vi "Main.vi"(9 "Test Titel":string, 10 "Cluster 2":T1={"Test Titel"="", "Test Type "="", "Project Number"="NA", "Unit Family"="Package", "Test Procedure #"="", "Data Collection Rate (HZ)"="", "Cluster"={" Pressure /Torque/ LVDT"={"Boolean"=FALSE, "Boolean 2"=FALSE, "Boolean 3"=FALSE, "Boolean 4"=FALSE, "Boolean 5"=FALSE, "Boolean 6"=FALSE, "Boolean 7"=FALSE, "Boolean 8"=FALSE}, "Name of Channel"={"ch1"="", "ch1 2"="", "ch1 3"="", "ch1 4"="", "ch1 5"="", "ch1 6"="", "ch1 7"="", "ch1 8"=""}, "Create New Test"=FALSE, "Name of Channel 2"={"ch1"="", "ch1 2"="", "ch1 3"="", "ch1 4"="", "ch1 5"="", "ch1 6"="", "ch1 7"="", "ch1 8"="", "ch1 9"="", "ch1 10"="", "ch1 11"="", "ch1 12"="", "ch1 13"="", "ch1 14"="", "ch1 15"=""}, "MOD1 ThermoCouple"={"Boolean"=FALSE, "Boolean 2"=FALSE, "Boolean 3"=FALSE, "Boolean 4"=FALSE, "Boolean 5"=FALSE, "Boolean 6"=FALSE, "Boolean 7"=FALSE, "Boolean 8"=FALSE, "Boolean 9"=FALSE, "Boolean 10"=FALSE, "Boolean 11"=FALSE, "Boolean 12"=FALSE, "Boolean 13"=FALSE, "Boolean 14"=FALSE, "Boolean 15"=FALSE, "Boolean 16"=FALSE}, "Internal SFI sensor number"={"ch1"="", "ch1 2"="", "ch1 3"="", "ch1 4"="", "ch1 5"="", "ch1 6"="", "ch1 7"="", "ch1 8"=""}, "Internal SFI sensor number"={"ch1"="", "ch1 2"="", "ch1 3"="", "ch1 4"="", "ch1 5"="", "ch1 6"="", "ch1 7"="", "ch1 8"="", "ch1 9"="", "ch1 10"="", "ch1 11"="", "ch1 12"="", "ch1 13"="", "ch1 14"="", "ch1 15"=""}}, "Sensor Serial Num"="", "Calibration Due"=""}) -> ()   [LabVIEW 2024]
uses:
  States.ctl
  Global 1.vi
  Wave forms.vi
panel:
  out "appended array 3":dbl[](array[numeric])
  in  "Table Control":string[][](table)
  out "Symbol":string
  in  "Combo Box":string(combo)
  in  "Boolean 2":bool
  in  "Log Interval\n(seconds)":dbl=0.5 min=0.1 max=10.0 step=0.1
  in  "Hours to Show 2":dbl=0.05
  in  "stop":bool
  out "appended array":string[](array[string])
  out "Array 3":string[](array[string])
  out "Array 2":string[](array[string])
  in  "Array":dbl[](array[numeric])
  in  "Boolean":bool
  out "Last Event Time (sec)":i32
  out "Event Counter":i32
  in  "Tab Control":enum32{"Main Configuration", "Graphs Display"}(tab)
  out "Array 5":string[](array[string])
  out "Array 4":string[](array[string])
  in  "Settings Button":bool
  in  "Add paramter":bool
  in  "Select Parameter to ADD":string(combo)
  in  "Record Button":bool
  in  "end":bool caption="Pause Button 2"
  in  "Initial":bool caption="Pause Button"
  out "Waveform Graph":dbl[][](graph)
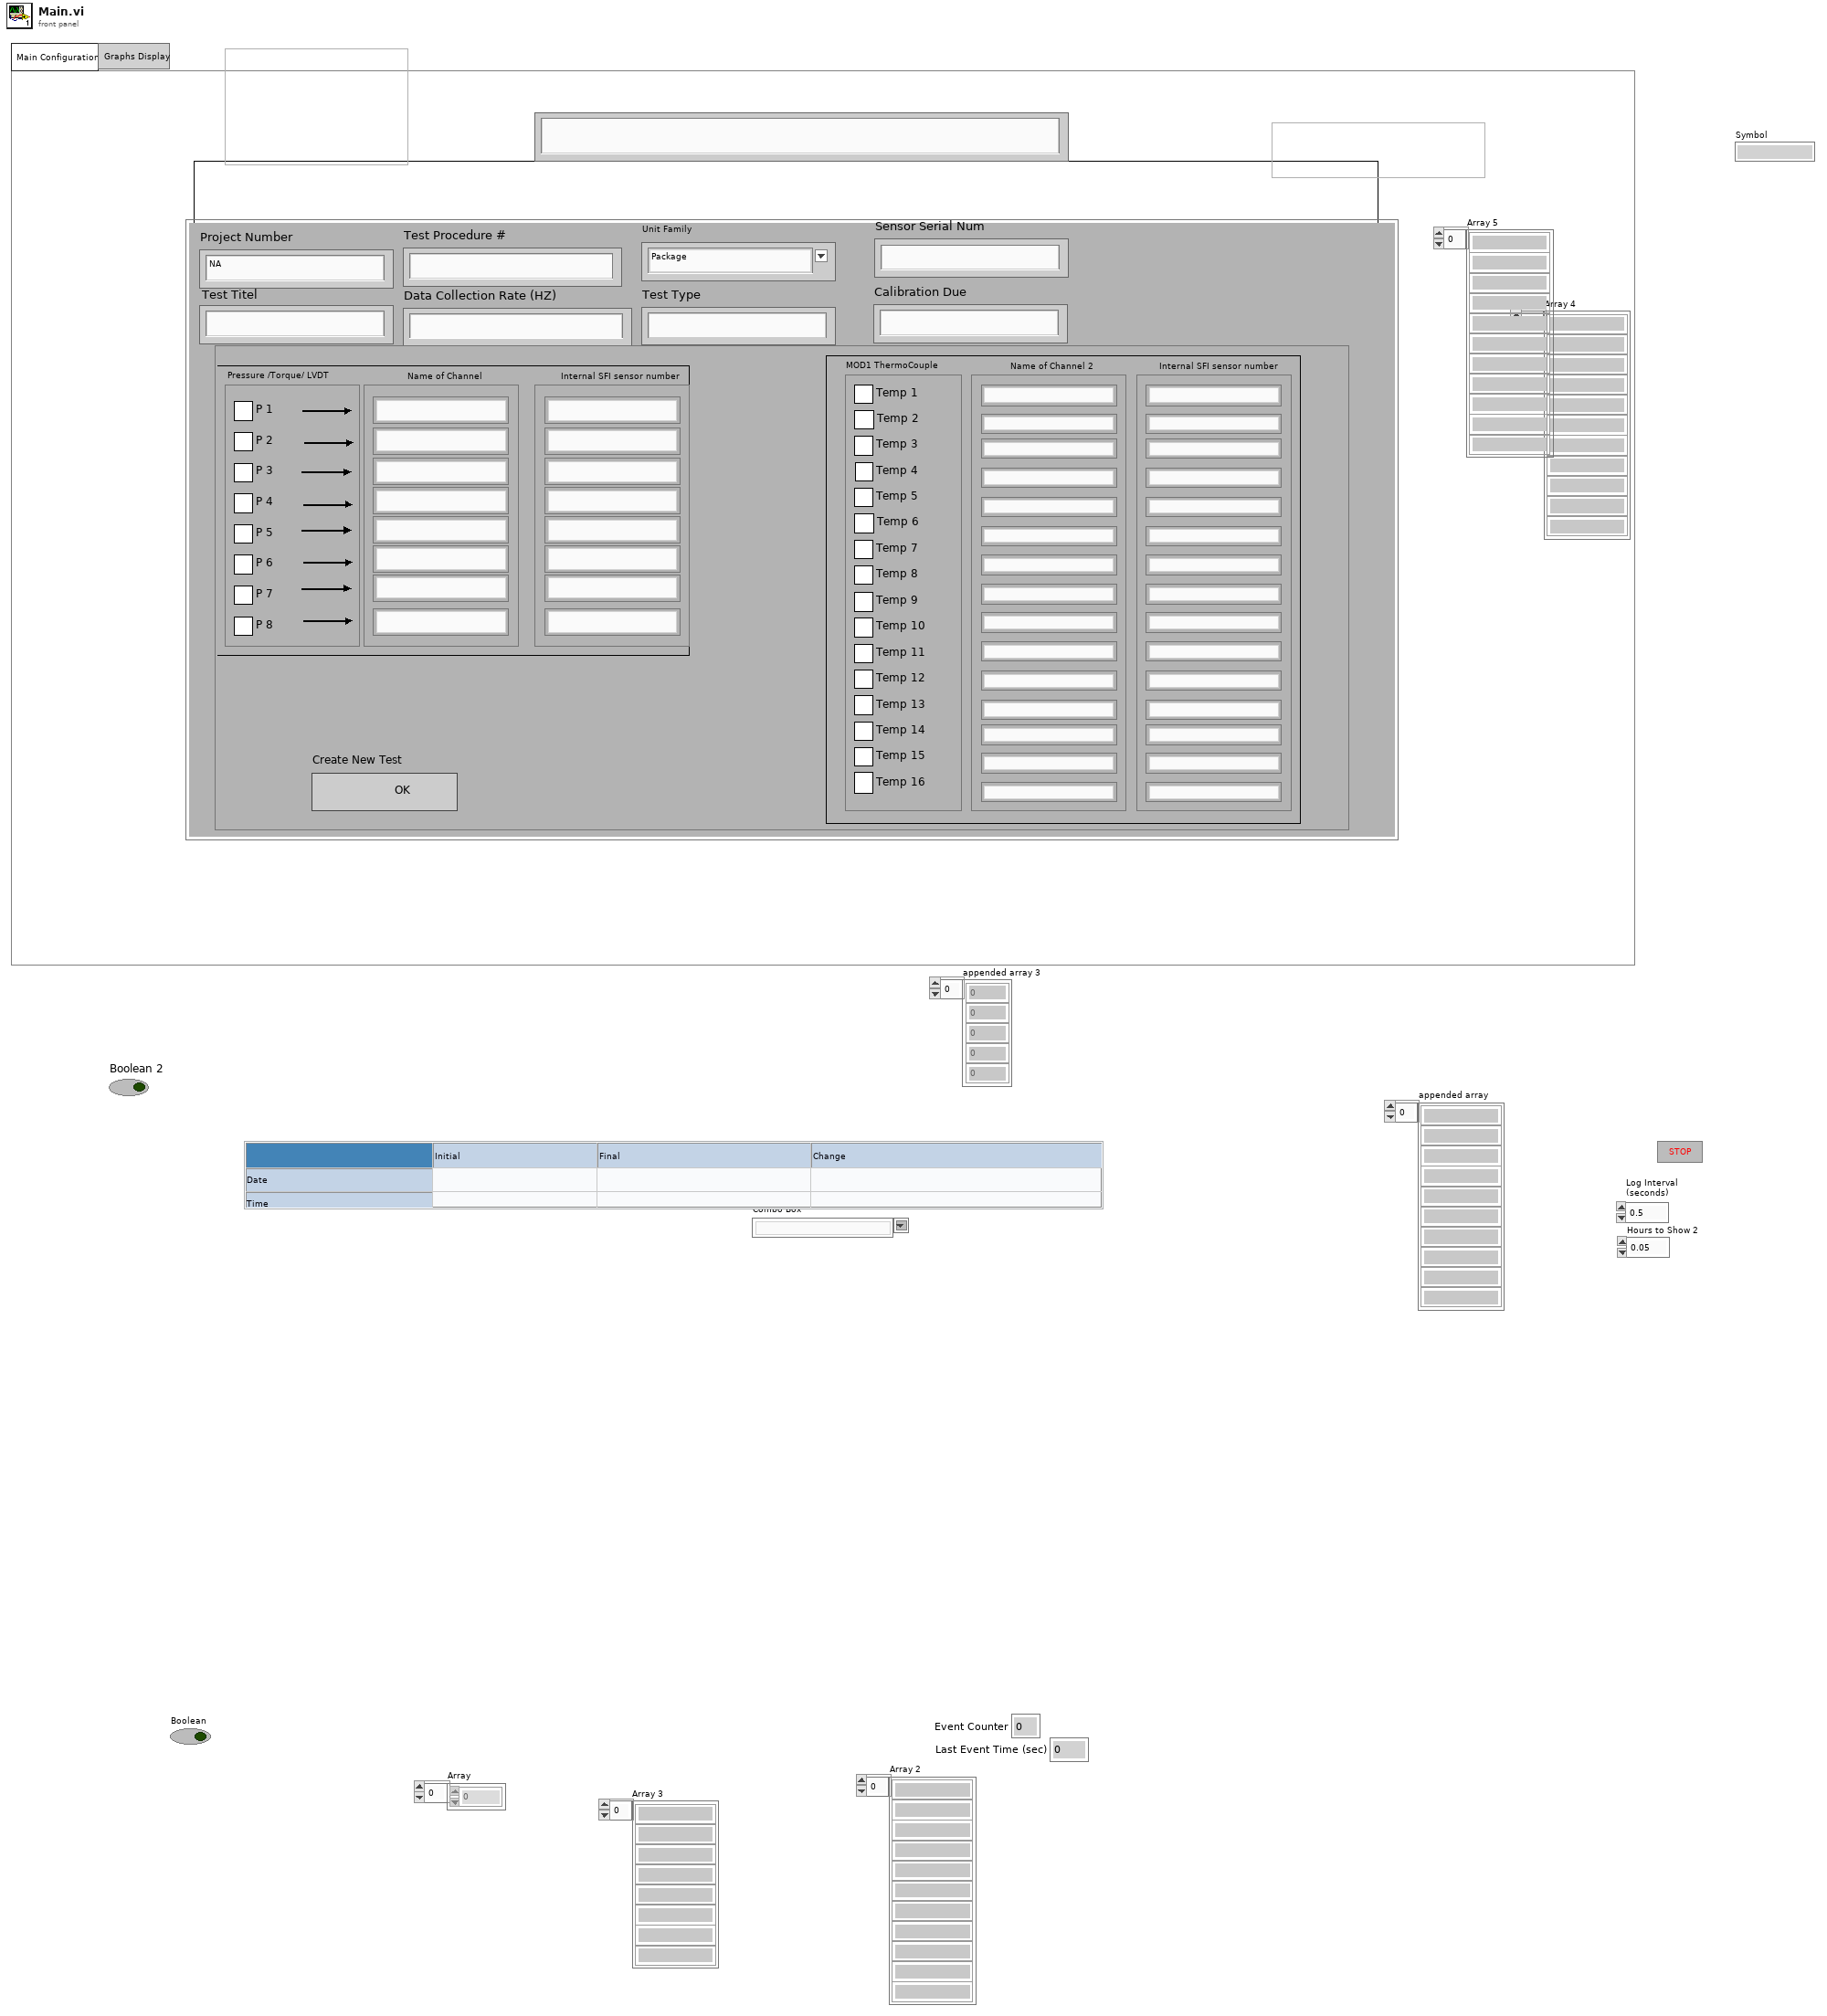
[diagram p1: front panel]
types:
  T1 = cluster{"Test Titel":string, "Test Type ":string, "Project Number":string, "Unit Family":string, "Test Procedure #":string, "Data Collection Rate (HZ)":string, "Cluster":cluster{" Pressure /Torque/ LVDT":cluster{"Boolean":bool, "Boolean 2":bool, "Boolean 3":bool, "Boolean 4":bool, "Boolean 5":bool, "Boolean 6":bool, "Boolean 7":bool, "Boolean 8":bool}, "Name of Channel":cluster{"ch1":string, "ch1 2":string, "ch1 3":string, "ch1 4":string, "ch1 5":string, "ch1 6":string, "ch1 7":string, "ch1 8":string}, "Create New Test":bool, "Name of Channel 2":cluster{"ch1":string, "ch1 2":string, "ch1 3":string, "ch1 4":string, "ch1 5":string, "ch1 6":string, "ch1 7":string, "ch1 8":string, "ch1 9":string, "ch1 10":string, "ch1 11":string, "ch1 12":string, "ch1 13":string, "ch1 14":string, "ch1 15":string}, "MOD1 ThermoCouple":cluster{"Boolean":bool, "Boolean 2":bool, "Boolean 3":bool, "Boolean 4":bool, "Boolean 5":bool, "Boolean 6":bool, "Boolean 7":bool, "Boolean 8":bool, "Boolean 9":bool, "Boolean 10":bool, "Boolean 11":bool, "Boolean 12":bool, "Boolean 13":bool, "Boolean 14":bool, "Boolean 15":bool, "Boolean 16":bool}, "Internal SFI sensor number":cluster{"ch1":string, "ch1 2":string, "ch1 3":string, "ch1 4":string, "ch1 5":string, "ch1 6":string, "ch1 7":string, "ch1 8":string}, "Internal SFI sensor number":cluster{"ch1":string, "ch1 2":string, "ch1 3":string, "ch1 4":string, "ch1 5":string, "ch1 6":string, "ch1 7":string, "ch1 8":string, "ch1 9":string, "ch1 10":string, "ch1 11":string, "ch1 12":string, "ch1 13":string, "ch1 14":string, "ch1 15":string}}, "Sensor Serial Num":string, "Calibration Due":string}
  T2 = typedef "States.ctl" = enum16{"Idel", "end test", "Selection", "Inittialize"}
  T3 = cluster{"Paramter":string, "Intital ":string, "Final":string, "Change":string, "Alarm Activate ":bool, "Symbol":string, "Value":string, "Alarm":bool}[]
  T4 = cluster{"Paramter":string, "Rate of Change":dbl, "X (sec)":dbl}[]
  T5 = cluster{"Paramter":string, "Intital ":string, "Final":string, "Change":string, "Alarm Activate ":bool, "Symbol":string, "Value":string, "Alarm":bool}
  T6 = cluster{"ch1":string, "ch1 2":string, "ch1 3":string, "ch1 4":string, "ch1 5":string, "ch1 6":string, "ch1 7":string, "ch1 8":string, "ch1 9":string, "ch1 10":string, "ch1 11":string, "ch1 12":string, "ch1 13":string, "ch1 14":string, "ch1 15":string}
  T7 = cluster{"Boolean":bool, "Boolean 2":bool, "Boolean 3":bool, "Boolean 4":bool, "Boolean 5":bool, "Boolean 6":bool, "Boolean 7":bool, "Boolean 8":bool, "Boolean 9":bool, "Boolean 10":bool, "Boolean 11":bool, "Boolean 12":bool, "Boolean 13":bool, "Boolean 14":bool, "Boolean 15":bool, "Boolean 16":bool}
  T8 = cluster{"Boolean":bool, "Boolean 2":bool, "Boolean 3":bool, "Boolean 4":bool, "Boolean 5":bool, "Boolean 6":bool, "Boolean 7":bool, "Boolean 8":bool}
  T9 = cluster{"ch1":string, "ch1 2":string, "ch1 3":string, "ch1 4":string, "ch1 5":string, "ch1 6":string, "ch1 7":string, "ch1 8":string}
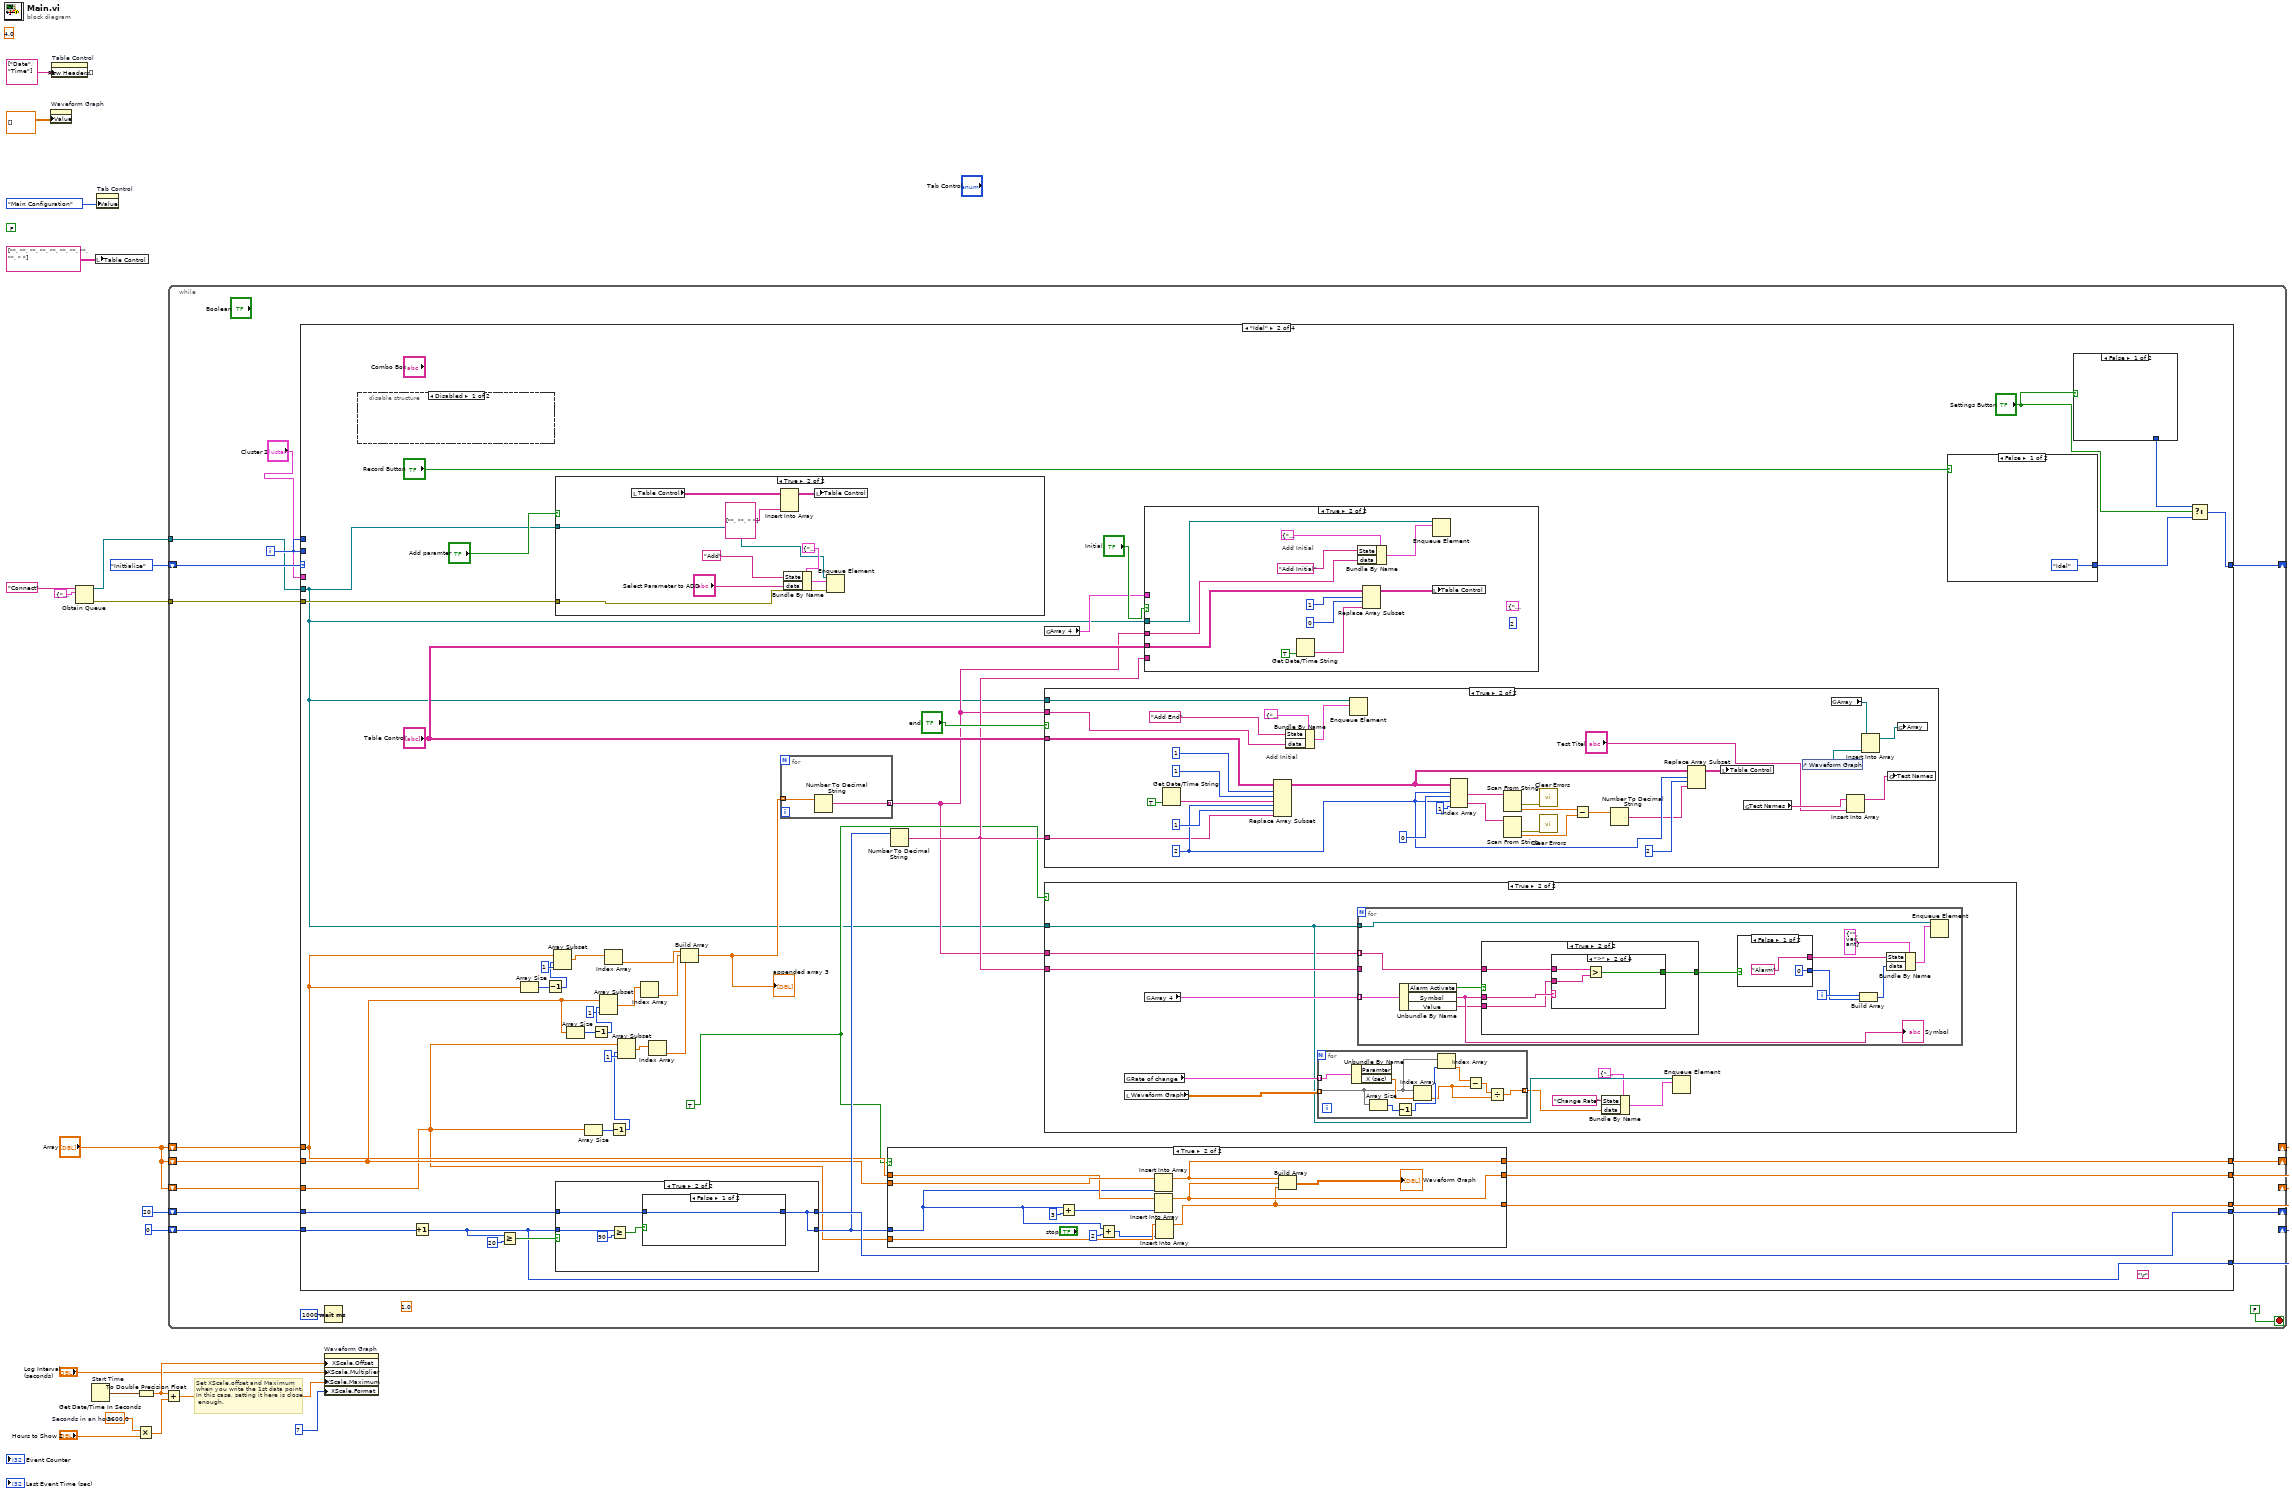
[diagram p0: block diagram]
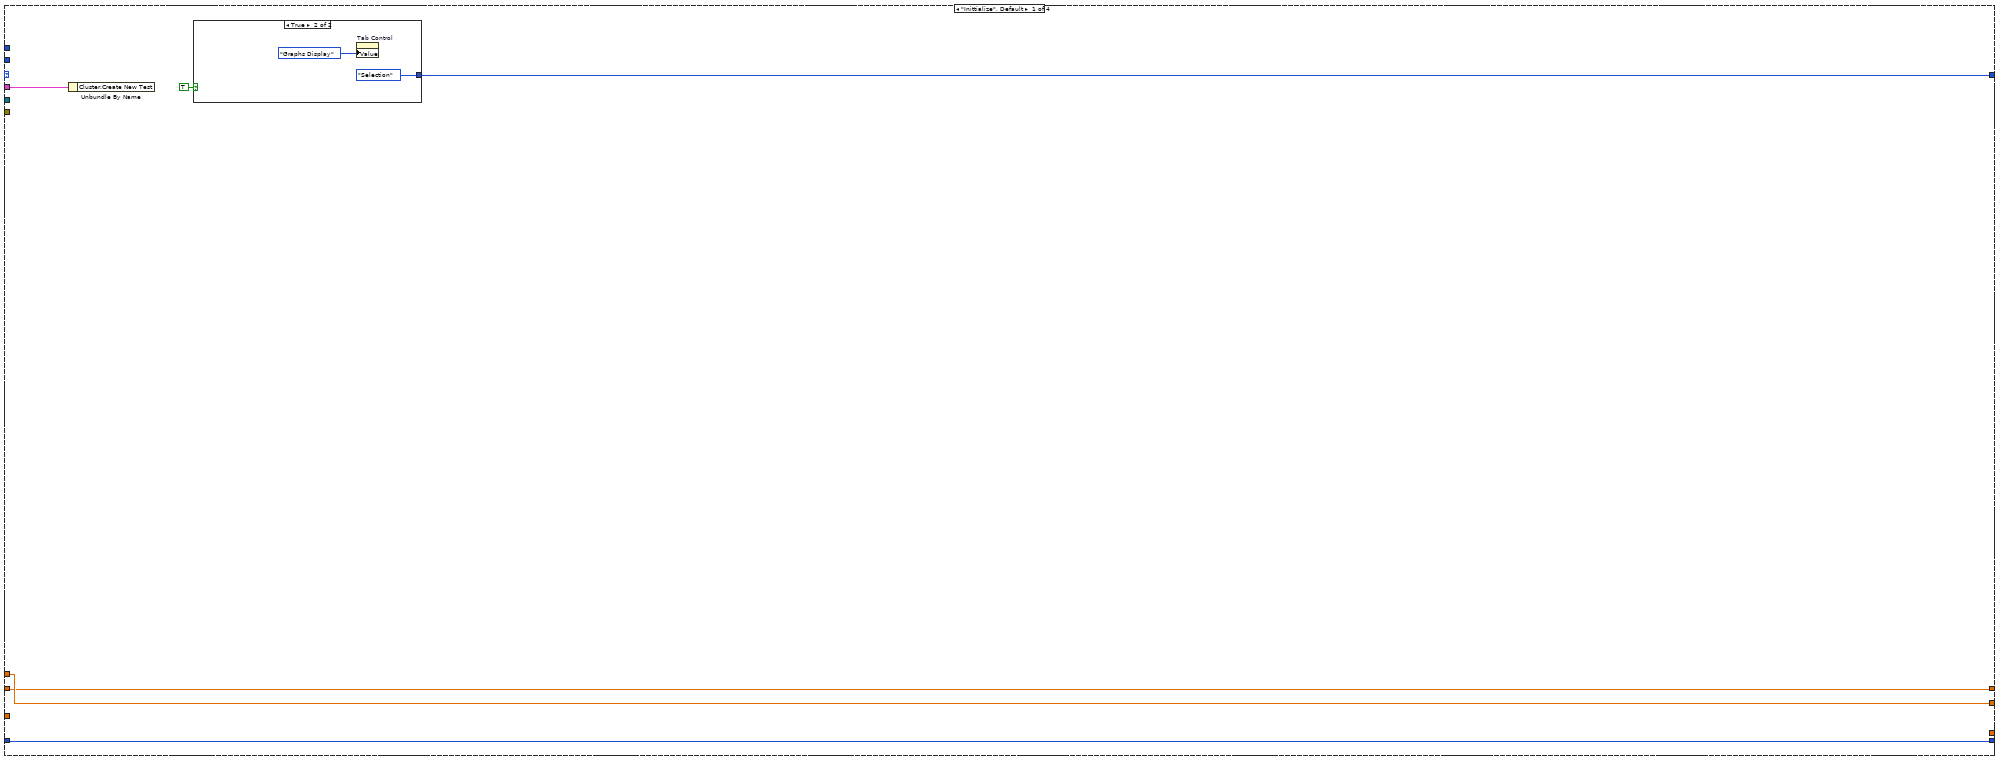
[diagram p2: hidden frame]
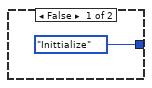
[diagram p3: hidden frame]
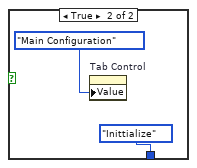
[diagram p4: hidden frame]
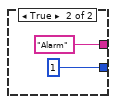
[diagram p6: hidden frame]
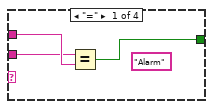
[diagram p8: hidden frame]
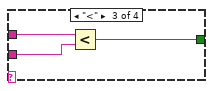
[diagram p9: hidden frame]
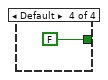
[diagram p10: hidden frame]
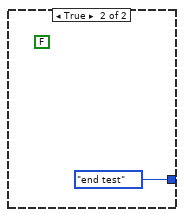
[diagram p12: hidden frame]
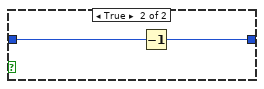
[diagram p17: hidden frame]
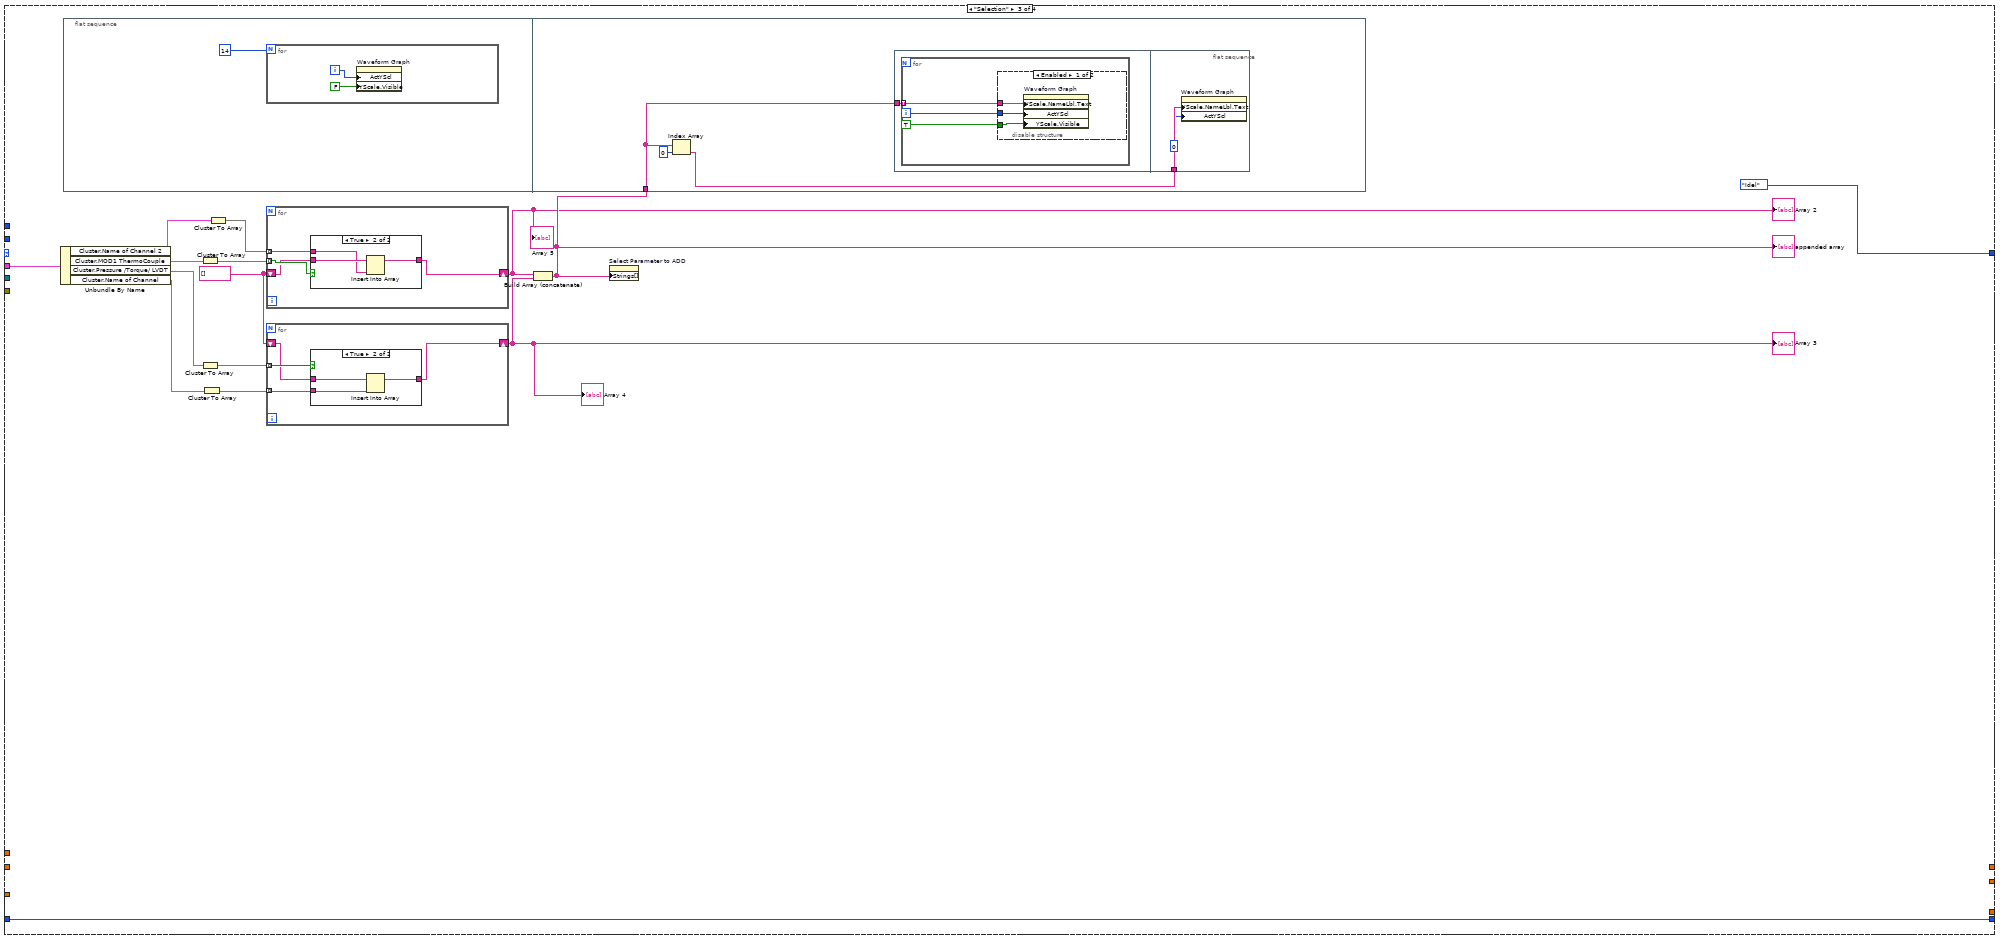
[diagram p19: hidden frame]
diagram:
  (unwired) 4.0
  (unwired) FALSE ("OK Button")
  w16 = 3600.0  # Seconds in an hour
  # "Set XScale.offset and Maximum\nwhen you write the 1st data point. \nIn this case, setting it here is close\n enough."
  n1 = property on="Waveform Graph" class="WFGraph (strict)"("Value"=dbl[][] [] ("Waveform Graph")) -> ()  [unwired: 2 in, 2 out]
  n2 = property on="Table Control" class="Tbl (strict)"("Row Headers[]"=string[] ["Date", "Time"] ("Row Header Strings[]")) -> ()  [unwired: 2 in, 2 out]
  n3 = Obtain Queue(name (unnamed)="Connect", element data type=cluster{"State":string, "data":variant} {"State"="", "data"=variant}) -> (queue out=w3:refnum<queue>, error out=w2:errorcluster)  [unwired: 3 in, 1 out]
  n4 = Get Date/Time In Seconds "Start Time"() -> (seconds since 1Jan1904=w17:timestamp)
  n5 = local write "Table Control"(string[][] [["", "", "", "", ""], ["", "", "", "", " "]] ("Test Results")) -> ()
  n6 = property on="Tab Control" class="TabCtl (strict)"("Value"=enum32{"Main Configuration", "Graphs Display"}."Main Configuration" ("Tab Control")) -> ()  [unwired: 2 in, 2 out]
  n7 = Multiply(x=w16, y="Hours to Show 2") -> (x*y=w18:dbl)
  n8 = To Double Precision Float(number=w17) -> (double precision float=w11:dbl)
  n9 = Add(x=w11, y=w18) -> (x+y=w9:dbl)
  n10 = while {
    shift-right: [w36] -> _
    shift-left: States."Inittialize" -> [w38]
    shift-right: [w33] -> _
    shift-left: "Array" -> [w34]
    shift-right: [w27] -> _
    shift-left: 20 -> [w31]
    shift-right: [w29] -> _
    shift-left: "Array" -> [w30]
    shift-right: [w26] -> _
    shift-left: 0 -> [w28]
    tunnel: w3 -> [w25]
    tunnel: w2 -> [w24]
    shift-right: [w22] -> _
    shift-left: "Array" -> [w23]
    i -> [w32]
    stop <- FALSE stop-if-true
    (unwired) 1.0 ("Log Interval\n(seconds)")
    n11 = case shown="\"Idel\"" w38 {
      tunnel: "Cluster 2" -> [w44 _ w239 _]
      tunnel: [w42 w72 States."Idel" States."end test"] -> w36
      tunnel: w34 -> [w40 w59 _ _]
      tunnel: w32 -> [_ _ _ _]
      tunnel: [w40 w91 _ _] -> w33
      tunnel: w32 -> [_ _ _ _]
      tunnel: [w43 w87 w228 _] -> w27
      tunnel: w31 -> [w43 w86 w228 _]
      tunnel: w30 -> [w41 w68 _ _]
      tunnel: [w41 w80 _ _] -> w29
      tunnel: w28 -> [_ w79 _ _]
      tunnel: [_ w78 _ _] -> w26
      tunnel: w25 -> [_ w48 _ _]
      tunnel: w24 -> [_ w76 _ _]
      tunnel: w23 -> [_ w58 _ _]
      tunnel: [_ w70 _ _] -> w22
      frame "Inittialize", Default {
        n12 = Unbundle By Name(w44) -> ()  [unwired: 1 out]
        n13 = case shown="True" TRUE {
          tunnel: [States."Inittialize" States."Selection"] -> w42
          frame False {
          }
          frame True {
            n14 = property on="Tab Control" class="TabCtl (strict)"("Value"=enum32{"Main Configuration", "Graphs Display"}."Graphs Display" ("Tab Control")) -> ()  [unwired: 2 in, 2 out]
          }
        }
      }
      frame "Idel" {
        w50 = TRUE ("Start Test")
        (unwired) "\r"
        n15 = disable-structure shown="Disabled" {
          frame Disabled {
          }
          frame Enabled {
          }
        }
        n16 = Increment(x=w79) -> (x+1=w78:i32)
        n17 = Greater Or Equal?(x=w78, y=20) -> (x >= y?=w88:bool)
        n18 = Array Size(array=w68) -> (size(s)=w67:i32)
        n19 = Decrement(x=w67) -> (x-1=w66:i32)
        n20 = Array Subset(array=w68, index=w66, length=1) -> (w57:dbl[])
        n21 = case shown="True" "Add paramter" {
          tunnel: w48 -> [_ w217]
          tunnel: w76 -> [_ w216]
          frame False {
          }
          frame True {
            n22 = local read "Table Control"() -> (w223:string[][])
            n23 = Insert Into Array(array=w223, new element=string[] ["", "", " "] ("new element/subarray")) -> (w222:string[][])  [unwired: 2 in]
            n24 = Bundle By Name(cluster=cluster{"State":string, "data":variant} {"State"="", "data"=variant}, "State"="Add", "data"="Select Parameter to ADD") -> (w220:cluster{"State":string, "data":variant})
            n25 = local write "Table Control"(w222) -> ()
            n26 = Enqueue Element(queue=w217, element=w220, error in (no error)=w216) -> ()  [unwired: 1 in, 3 out]
          }
        }
        n27 = case shown="True" w88 {
          tunnel: [w207 w211] -> w82
          tunnel: w78 -> [w207 w210]
          tunnel: [w206 w211] -> w87
          tunnel: w86 -> [w206 w212]
          frame False {
          }
          frame True {
            n28 = Greater Or Equal?(x=w210, y=90) -> (x >= y?=w208:bool)
            n29 = case shown="False" w208 {
              tunnel: w212 -> [w213 w215]
              tunnel: [w213 w214] -> w211
              frame False {
              }
              frame True {
                n30 = Decrement(x=w215) -> (x-1=w214:i32)
              }
            }
          }
        }
        n31 = Array Size(array=w59) -> (size(s)=w64:i32)
        n32 = Array Size(array=w58) -> (size(s)=w61:i32)
        n33 = Decrement(x=w64) -> (x-1=w65:i32)
        n34 = Array Subset(array=w59, index=w65, length=1) -> (w56:dbl[])
        n35 = Index Array(array=w57) -> (element=w54:dbl)  [unwired: 1 in]
        n36 = Decrement(x=w61) -> (x-1=w60:i32)
        n37 = Array Subset(array=w58, index=w60, length=1) -> (w55:dbl[])
        n38 = Index Array(array=w56) -> (element=w53:dbl)  [unwired: 1 in]
        n39 = Index Array(array=w55) -> (element=w52:dbl)  [unwired: 1 in]
        n40 = Build Array(w54, w53, w52) -> (w51:dbl[])
        "appended array 3" <- w51
        n41 = for {
          tunnel: w51 -> [w95] mode=indexing
          tunnel: [w94] -> w49 mode=indexing
          n42 = Number To Decimal String(number=w95) -> (decimal integer string=w94:string)  [unwired: 1 in]
        }
        n43 = case shown="True" w50 {
          tunnel: w59 -> [w193 w205]
          tunnel: [w193 w204] -> w91
          tunnel: w82 -> [_ w196]
          tunnel: w68 -> [w192 w202]
          tunnel: [w192 w200] -> w80
          tunnel: w58 -> [w191 w198]
          tunnel: [w191 w194] -> w70
          frame False {
          }
          frame True {
            n44 = Add(x=w196, y=3) -> (x+y=w201:i32)
            n45 = Add(x=w196, y=2) -> (x+y=w195:i32)
            n46 = Insert Into Array(array=w205, new element=w196) -> (w204:dbl[])  [unwired: 1 in]
            n47 = Insert Into Array(array=w202, new element=w201) -> (w200:dbl[])  [unwired: 1 in]
            n48 = Insert Into Array(array=w198, new element=w195) -> (w194:dbl[])  [unwired: 1 in]
            n49 = Build Array(w204, w200, w194) -> (→"Waveform Graph":dbl[][])
          }
        }
        n50 = Number To Decimal String(number=w82) -> (decimal integer string=w75:string)  [unwired: 1 in]
        n51 = global read "Global 1.vi" "Array 4"() -> (w77:T3)
        n52 = case shown="True" "end" {
          tunnel: "Table Control" -> [_ w178]
          tunnel: w75 -> [_ w155]
          tunnel: w48 -> [_ w159]
          tunnel: w49 -> [_ w154]
          frame False {
          }
          frame True {
            w165 = 2 ("index (row)")
            # "Add Initial"
            n53 = Get Date/Time String(want seconds? (F)=TRUE ("UTC format")) -> (time string=w175:string)  [unwired: 2 in, 1 out]
            n54 = Replace Array Subset(array=w178, new element #1=w175, index (row) #1=1 ("index (row)"), index (col) #1=1 ("disabled index (col)"), new element #2=w155, index (row) #2=w165, index (col) #2=1 ("disabled index (col)")) -> (w167:string[][])
            n55 = Bundle By Name(cluster=cluster{"State":string, "data":variant} {"State"="", "data"=variant}, "State"="Add End", "data"=w154) -> (w156:cluster{"State":string, "data":variant})
            n56 = Enqueue Element(queue=w159, element=w156) -> ()  [unwired: 2 in, 3 out]
            n57 = Index Array(array=w167, index (row) #1=w165, index (col) #1=0 ("disabled index (col)"), index (row) #2=w165, index (col) #2=1 ("index (col)")) -> (element #1=w171:string, element #2=w170:string)
            n58 = Scan From String(input string=w171) -> (error out=w161:errorcluster, output 1=w169:dbl)  [unwired: 4 in, 2 out]
            n59 = Scan From String(input string=w170) -> (error out=w160:errorcluster, output 1=w168:dbl)  [unwired: 4 in, 2 out]
            n60 = call <vilib>:"Clear Errors.vi"("error in (no error)"=w161) -> ()  [unwired: 5 in, 2 out]
            n61 = call <vilib>:"Clear Errors.vi"("error in (no error)"=w160) -> ()  [unwired: 5 in, 2 out]
            n62 = Subtract(x=w169, y=w168) -> (x-y=w163:dbl)
            n63 = Number To Decimal String(number=w163) -> (decimal integer string=w162:string)  [unwired: 1 in]
            n64 = Replace Array Subset(array=w167, new element=w162, index (row)=w165, index (col)=2 ("disabled index (col)")) -> (w166:string[][])
            n65 = local write "Table Control"(w166) -> ()
            n66 = global read "Wave forms.vi" "Test Names"() -> (w150:string[])
            n67 = control-ref of="Waveform Graph"() -> (w152:refnum<vi>)
            n68 = global read "Wave forms.vi" "Array"() -> (w151:refnum<vi>[])
            n69 = Insert Into Array(array=w150, new element="Test Titel") -> (w149:string[])  [unwired: 1 in]
            n70 = Insert Into Array(array=w151, new element=w152) -> (w153:refnum<vi>[])  [unwired: 1 in]
            n71 = global write "Wave forms.vi" "Test Names"(w149) -> ()
            n72 = global write "Wave forms.vi" "Array"(w153) -> ()
          }
        }
        n73 = case shown="True" w50 {
          tunnel: w75 -> [_ w104]
          tunnel: w48 -> [_ w101]
          tunnel: w49 -> [_ w96]
          frame False {
          }
          frame True {
            n74 = global read "Global 1.vi" "Rate of change"() -> (w103:T4)
            n75 = local read "Waveform Graph"() -> (w102:dbl[][])
            n76 = global read "Global 1.vi" "Array 4"() -> (w105:T3)
            n77 = for {
              tunnel: w103 -> [w114] mode=indexing
              tunnel: w102 -> [w112] mode=indexing
              tunnel: [w106] -> w98 mode=indexing
              n78 = Unbundle By Name(w114) -> ("X (sec)"=w113:dbl)  [unwired: 1 out]
              n79 = Array Size(array=w112) -> (size(s)=w111:i32)
              n80 = Decrement(x=w111) -> (x-1=w110:i32)
              n81 = Index Array(array=w112, index=w113) -> (element=w107:dbl)
              n82 = Index Array(array=w112, index=w110) -> (element=w109:dbl)
              n83 = Subtract(x=w109, y=w107) -> (x-y=w108:dbl)
              n84 = Divide(x=w108, y=w107) -> (x/y=w106:dbl)
            }
            n85 = for {
              tunnel: w105 -> [w127] mode=indexing
              tunnel: w104 -> [_]
              tunnel: w101 -> [w121]
              tunnel: w96 -> [w118] mode=indexing
              i -> [w117]
              n86 = Unbundle By Name(w127) -> ("Alarm Activate"=w126:bool, "Symbol"=w125:string, "Value"=w124:string)
              "Symbol" <- w125
              n87 = case shown="True" w126 {
                tunnel: w125 -> [_ w135]
                tunnel: w124 -> [_ w134]
                tunnel: w118 -> [_ w133]
                tunnel: [_ w132] -> w122
                frame False {
                }
                frame True {
                  n88 = case shown="\">\"" w135 {
                    tunnel: w134 -> [w137 w139 w142 _]
                    tunnel: w133 -> [w138 w140 w143 _]
                    tunnel: [w136 w141 w144 FALSE] -> w132
                    frame "=" {
                      (unwired) "Alarm" ("State")
                      n89 = Equal?(x=w137, y=w138) -> (x = y?=w136:bool)
                    }
                    frame ">" {
                      n90 = Greater?(x=w140, y=w139) -> (0:w141:bool)
                    }
                    frame "<" {
                      n91 = Less?(x=w143, y=w142) -> (x < y?=w144:bool)
                    }
                    frame Default {
                    }
                  }
                }
              }
              n92 = case shown="False" w122 {
                tunnel: ["Alarm" ("State") "Alarm" ("State")] -> w123
                tunnel: [0 ("element") 1 ("element")] -> w116
                frame False {
                }
                frame True {
                }
              }
              n93 = Build Array(w117, w116) -> (w115:i32[])
              n94 = Bundle By Name(cluster=cluster{"State":string, "data":variant} {"State"="", "data"=variant} ("element"), "State"=w123, "data"=w115) -> (w119:cluster{"State":string, "data":variant})
              n95 = Enqueue Element(queue=w121, element=w119) -> ()  [unwired: 2 in, 3 out]
            }
            n96 = Bundle By Name(cluster=cluster{"State":string, "data":variant} {"State"="", "data"=variant} ("input cluster"), "State"="Change Rate", "data"=w98) -> (w97:cluster{"State":string, "data":variant})
            n97 = Enqueue Element(queue=w101, element=w97) -> ()  [unwired: 2 in, 3 out]
          }
        }
        n98 = case shown="True" "Initial" {
          tunnel: "Table Control" -> [_ w190]
          tunnel: w75 -> [_ _]
          tunnel: w77 -> [_ _]
          tunnel: w48 -> [_ w184]
          tunnel: w49 -> [_ w180]
          frame False {
          }
          frame True {
            (unwired) T5 {"Paramter"="", "Intital "="", "Final"="", "Change"="", "Alarm Activate "=FALSE, "Symbol"="", "Value"="", "Alarm"=FALSE} ("new element/subarray")
            (unwired) 2 ("index (row)")
            # "Add Initial"
            n99 = Get Date/Time String(want seconds? (F)=TRUE ("UTC format")) -> (time string=w185:string)  [unwired: 2 in, 1 out]
            n100 = Bundle By Name(cluster=cluster{"State":string, "data":variant} {"State"="", "data"=variant}, "State"="Add Initial", "data"=w180) -> (w182:cluster{"State":string, "data":variant})
            n101 = Replace Array Subset(array=w190, new element=w185, index (row)=1, index (col)=0 ("disabled index (col)")) -> (w188:string[][])
            n102 = Enqueue Element(queue=w184, element=w182) -> ()  [unwired: 2 in, 3 out]
            n103 = local write "Table Control"(w188) -> ()
          }
        }
        n104 = case shown="False" "Record Button" {
          tunnel: [States."Idel" States."end test"] -> w73
          frame False {
          }
          frame True {
            (unwired) FALSE ("OK Button")
          }
        }
        n105 = case shown="False" "Settings Button" {
          tunnel: [_ States."Inittialize"] -> w71
          frame False {
          }
          frame True {
            n106 = property on="Tab Control" class="TabCtl (strict)"("Value"=enum32{"Main Configuration", "Graphs Display"}."Main Configuration" ("Tab Control")) -> ()  [unwired: 2 in, 2 out]
          }
        }
        n107 = Select(t=w71, s="Settings Button", f=w73) -> (s? t:f=w72:T2)
      }
      frame "Selection" {
        w230 = string[] []
        n108 = Unbundle By Name(w239) -> ("Cluster.Name of Channel 2"=w234:T6, "Cluster.MOD1 ThermoCouple"=w238:T7, "Cluster.Pressure /Torque/ LVDT"=w237:T8, "Cluster.Name of Channel"=w232:T9)
        n109 = flat-sequence {
          tunnel: w229 -> [w245]
          frame #0 {
            n110 = for {
              N: 14 -> [_]
              i -> [w242]
              n111 = property on="Waveform Graph" class="WFGraph (strict)"("ActYScl"=w242, "YScale.Visible"=FALSE ("Y Scale.Visible")) -> ()  [unwired: 2 in, 2 out]
            }
          }
          frame #1 {
            n112 = Index Array(array=w245, index=0) -> (element=w243:string)
            n113 = flat-sequence {
              tunnel: w245 -> [w246]
              tunnel: w243 -> [w254]
              frame #0 {
                n114 = for {
                  tunnel: w246 -> [w249] mode=indexing
                  i -> [w248]
                  n115 = disable-structure shown="Enabled" {
                    disable-tunnel: w249 -> [w252 _]
                    disable-tunnel: w248 -> [w251 _]
                    disable-tunnel: TRUE ("Y Scale.Visible") -> [w250 _]
                    frame Enabled {
                      n116 = property on="Waveform Graph" class="WFGraph (strict)"("YScale.NameLbl.Text"=w252, "ActYScl"=w251, "YScale.Visible"=w250) -> ()  [unwired: 2 in, 2 out]
                    }
                    frame Disabled {
                    }
                  }
                }
              }
              frame #1 {
                n117 = property on="Waveform Graph" class="WFGraph (strict)"("YScale.NameLbl.Text"=w254, "ActYScl"=0 ("Active Y Scale")) -> ()  [unwired: 2 in, 2 out]
              }
            }
          }
        }
        n118 = Cluster To Array(cluster=w238) -> (array=w236:bool[])
        n119 = Cluster To Array(cluster=w237) -> (array=w235:bool[])
        n120 = Cluster To Array(cluster=w232) -> (array=w231:string[])
        n121 = Cluster To Array(cluster=w234) -> (array=w233:string[])
        n122 = for {
          tunnel: w236 -> [w266] mode=indexing
          tunnel: w233 -> [w263] mode=indexing
          shift-right: [w264] -> w226
          shift-left: w230 -> [w265]
          n123 = case shown="True" w266 {
            tunnel: w265 -> [w267 w270]
            tunnel: [w267 w269] -> w264
            tunnel: w263 -> [_ w268]
            frame False {
            }
            frame True {
              n124 = Insert Into Array(array=w270, new element=w268) -> (w269:string[])  [unwired: 1 in]
            }
          }
        }
        "Array 2" <- w226
        "Array 5" <- w226
        n125 = for {
          tunnel: w235 -> [w258] mode=indexing
          tunnel: w231 -> [w257] mode=indexing
          shift-right: [w255] -> w227
          shift-left: w230 -> [w256]
          n126 = case shown="True" w258 {
            tunnel: w256 -> [w259 w262]
            tunnel: [w259 w261] -> w255
            tunnel: w257 -> [_ w260]
            frame False {
            }
            frame True {
              n127 = Insert Into Array(array=w262, new element=w260) -> (w261:string[])  [unwired: 1 in]
            }
          }
        }
        "Array 3" <- w227
        "Array 4" <- w227
        n128 = Build Array (concatenate)(w226, w227) -> (w229:string[])
        "appended array" <- w229
        n129 = property on="Select Parameter to ADD" class="CmbBox"("Strings[]"=w229) -> ()  [unwired: 2 in, 2 out]
      }
      frame "end test" {
        n130 = case shown="True" "Boolean 2" {
          frame False {
          }
          frame True {
          }
        }
      }
    }
    n131 = Wait (ms)(milliseconds to wait=u32 1000) -> ()  [unwired: 1 out]
  }
  n132 = property on="Waveform Graph" class="WFGraph (strict)"("XScale.Offset"=w11, "XScale.Multiplier"="Log Interval\n(seconds)", "XScale.Maximum"=w9, "XScale.Format"=u8 7 ("X Scale.Display Format:Format")) -> ()  [unwired: 2 in, 2 out]
